vi "Remove_zeros.vi"(11 "Float_char":string="c") -> (3 "float_adaptive":string)   [LabVIEW 2025, in "Procotol_class.lvclass"]
uses:
  Procotol_class.lvclass
  <vilib>/regexp/Match Regular Expression.xnode
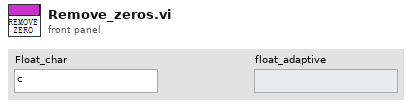
[diagram p1: front panel]
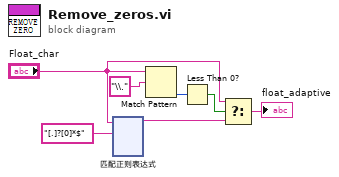
[diagram p0: block diagram]
diagram:
  n1 = xnode "匹配正则表达式"("输入字符串"="Float_char", "正则表达式"="[.]?[0]*$") -> ("匹配之前"=w2:string)  [unwired: 4 in, 4 out]
  n2 = Match Pattern(string="Float_char", regular expression="\\." ("正则表达式")) -> (offset past match=w5:i32)  [unwired: 1 in, 3 out]
  n3 = Less Than 0?(x=w5) -> (x < 0?=w4:bool)
  n4 = Select(t="Float_char", s=w4, f=w2) -> (s? t:f=→"float_adaptive":string)
